vi "FuncVI-Rad.vi"(5 "InstanceRef":T2, 9 "arg list":T1[](array[typedef]) {"num" format="%.2f"}) -> (0 "error out":bool, 3 "result":T1 {"num" format="%.2f"})   [LabVIEW 2021]
doc: "::: CalcExpress Toolkit :::\nCopyright (c) 2000-2026 Konstantin Shifershteyn. All rights reserved."
uses:
  cetypes.llb/CalcExpress Function Argument Info.ctl
  cetypes.llb/CalcExpress Instance RefNum.ctl
panel:
  in  "max arg num":i32=1
  in  "min arg num":i32=1
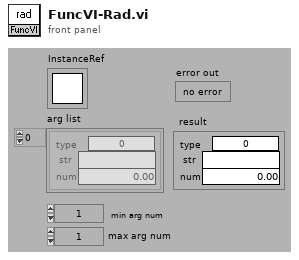
[diagram p1: front panel]
types:
  T1 = typedef "CalcExpress Function Argument Info.ctl" = cluster{"type":u32, "str":string, "num":dbl}
  T2 = typedef "CalcExpress Instance RefNum.ctl" = refnum<k1>
  T3 = enum16{"DBL scalar", "CDB scalar", "DBL array", "CDB array", "ERROR"}
  T4 = typedef "CalcExpress Data Type.ctl" = enum32{"String", "DBL Number", "identifier", "1D Array of DBL", "2D Array of DBL", "CDB Number", "1D Array of CDB", "2D Array of CDB", "1D Array of String", "2D Array of String", "Unknown data type"}
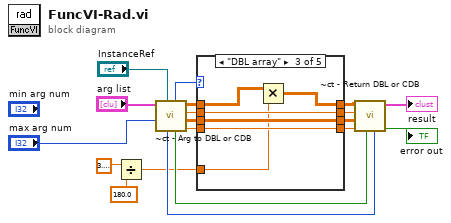
[diagram p0: block diagram]
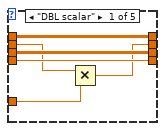
[diagram p2: hidden frame]
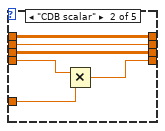
[diagram p3: hidden frame]
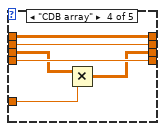
[diagram p4: hidden frame]
diagram:
  n1 = Divide(x=3.141592653589793, y=180.0) -> (x/y=w2:dbl)
  n2 = call "~ct - Arg to DBL or CDB.vi"("InstanceRef"="InstanceRef", "max args"="max arg num", "args list"="arg list") -> ("CDB"=w12:cdb, "2D CDB"=w13:cdb[][], "DBL"=w11:dbl, "2D DBL"=w10:dbl[][], "error out"=w15:bool, "category"=w5:T3, "arg type"=w14:T4)  [unwired: 2 in]
  n3 = case shown="\"DBL array\"" w5 {
    tunnel: w13 -> [w24 w30 w37 w39 w44]
    tunnel: w12 -> [w23 w27 w36 w42 w45]
    tunnel: w11 -> [w21 w29 w35 w41 w46]
    tunnel: w10 -> [w25 w31 w33 w43 w47]
    tunnel: [w25 w31 w34 w43 w47] -> w9
    tunnel: [w22 w29 w35 w41 w46] -> w8
    tunnel: [w24 w30 w37 w40 w44] -> w7
    tunnel: [w23 w28 w36 w42 w45] -> w6
    tunnel: w2 -> [w20 w26 w32 w38 _]
    frame "DBL scalar" {
      n4 = Multiply(x=w21, y=w20) -> (x*y=w22:dbl)
    }
    frame "CDB scalar" {
      n5 = Multiply(x=w27, y=w26) -> (x*y=w28:cdb)
    }
    frame "DBL array" {
      n6 = Multiply(x=w33, y=w32) -> (x*y=w34:dbl[][])
    }
    frame "CDB array" {
      n7 = Multiply(x=w39, y=w38) -> (x*y=w40:cdb[][])
    }
    frame "ERROR" {
    }
  }
  n8 = call "~ct - Return DBL or CDB.vi"("type"=w14, "error in"=w15, "CDB"=w6, "2D CDB"=w7, "DBL"=w8, "2D DBL"=w9) -> ("error out"=→"error out":bool, "result"=→"result":T1)  [unwired: 4 in]
